vi "text_transceiver_sim.vi"() -> ()   [LabVIEW 2024]
uses:
  <vilib>/addons/Modulation/Digital/Channel Coding/MT Convolutional Encoder (Rate).vi
  <vilib>/Analysis/2dsp.llb/Inverse Complex FFT.vi
  <vilib>/Analysis/2dsp.llb/Complex FFT.vi
  <vilib>/addons/Modulation/Digital/Support/Common/Validators/mod_Generate Bits Validate.vi
  <vilib>/addons/Modulation/Digital/General/subVIs/mod_Generate Bits Pattern.vi
  <vilib>/addons/Modulation/Analog/support/mod_Set Error Source.vi
  <vilib>/addons/Modulation/Digital/Support/Common/Validators/mod_Validate Bit Stream.vi
  <vilib>/addons/Modulation/Digital/Channel Coding/Convolutional codes/mod_Convolutional encoder.vi
  <vilib>/addons/Modulation/Digital/Support/Common/Validators/mod_Validate Number of Rows Columns.vi
  <vilib>/addons/Modulation/Digital/Channel Coding/Block codes/subVIs/mod_Buffer block code info.vi
  <vilib>/addons/Modulation/Digital/Interleaving/Block Interleaver/mod_Block Interleaver (Matrix).vi
  <vilib>/addons/Modulation/Digital/DeInterleaving/Block DeInterleaver/mod_Block DeInterleaver (Matrix).vi
  <vilib>/addons/Modulation/Digital/Channel Coding/Convolutional codes/subVIs/mod_Generate encoder tap connections.vi
  <vilib>/addons/Modulation/Digital/Channel Coding/Convolutional codes/subVIs/mod_Perform convolutional encoding.vi
  <vilib>/addons/Modulation/Digital/Channel Coding/Block codes/subVIs/mod_Buffer block code info (I8).vi
  <vilib>/addons/Modulation/Digital/Channel Coding/Convolutional codes/subVIs/mod_Generate valid reset (convolutional, I8).vi
  <vilib>/addons/Modulation/Digital/Channel Coding/Convolutional codes/subVIs/mod_Select known generator matrix.vi
  <vilib>/addons/Modulation/Digital/Support/Common/Validators/mod_Validate Convolutional Encoder prms.vi
  <vilib>/addons/Modulation/Digital/General/MT Map Bits to PSK Symbols.vi
  <vilib>/addons/Modulation/Digital/General/subVIs/mod_Generate Bits PN Sequence.vi
  <vilib>/addons/Modulation/Digital/General/MT Map Bits to QAM Symbols.vi
  <vilib>/addons/Modulation/Digital/General/MT Map PSK Symbols to Bits.vi
  <vilib>/addons/Modulation/Digital/Channel Coding/MT Convolutional Decoder (Viterbi Hard Decision, Rate).vi
  <vilib>/addons/Modulation/Digital/General/MT Map QAM Symbols to Bits.vi
  <vilib>/Analysis/NI_AALPro.lvlib
  <vilib>/addons/Modulation/niDMT.lvlib
panel:
  in  "Ts":dbl
  out "x*y 3":cdb[](array[numeric])
  out "Coarse estimate":dbl
  out "Fine freq est":dbl
  in  "Delay":i32
  in  "freq_offset":dbl
  out "coarse freq est":dbl
  out "Fine estimate":i32
  out "Wifi signal":cdb[](array[numeric])
  out "Wifi signal after coarse freq sync":cdb[](array[numeric])
  out "Channel Estimate":cdb[](array[numeric])
  out "Received Message":string
  out "message bitstream":i8[](array[numeric])
  out "Header and payload symbols concetanated":cdb[][](array[numeric])
  out "Pilot polarities":dbl[][](array[numeric])
  out "Header symbols":cdb[](array[numeric]) format="%.3f"
  out "0, 1":i16
  in  "bit order":enum16{"MSB first", "LSB first"}(ring)=enum."LSB first"
  out "Message Length (bits)":i32
  in  "text message":string
  out "LLTF":cdb[](array[numeric])
  out "LSTF":cdb[](array[numeric])
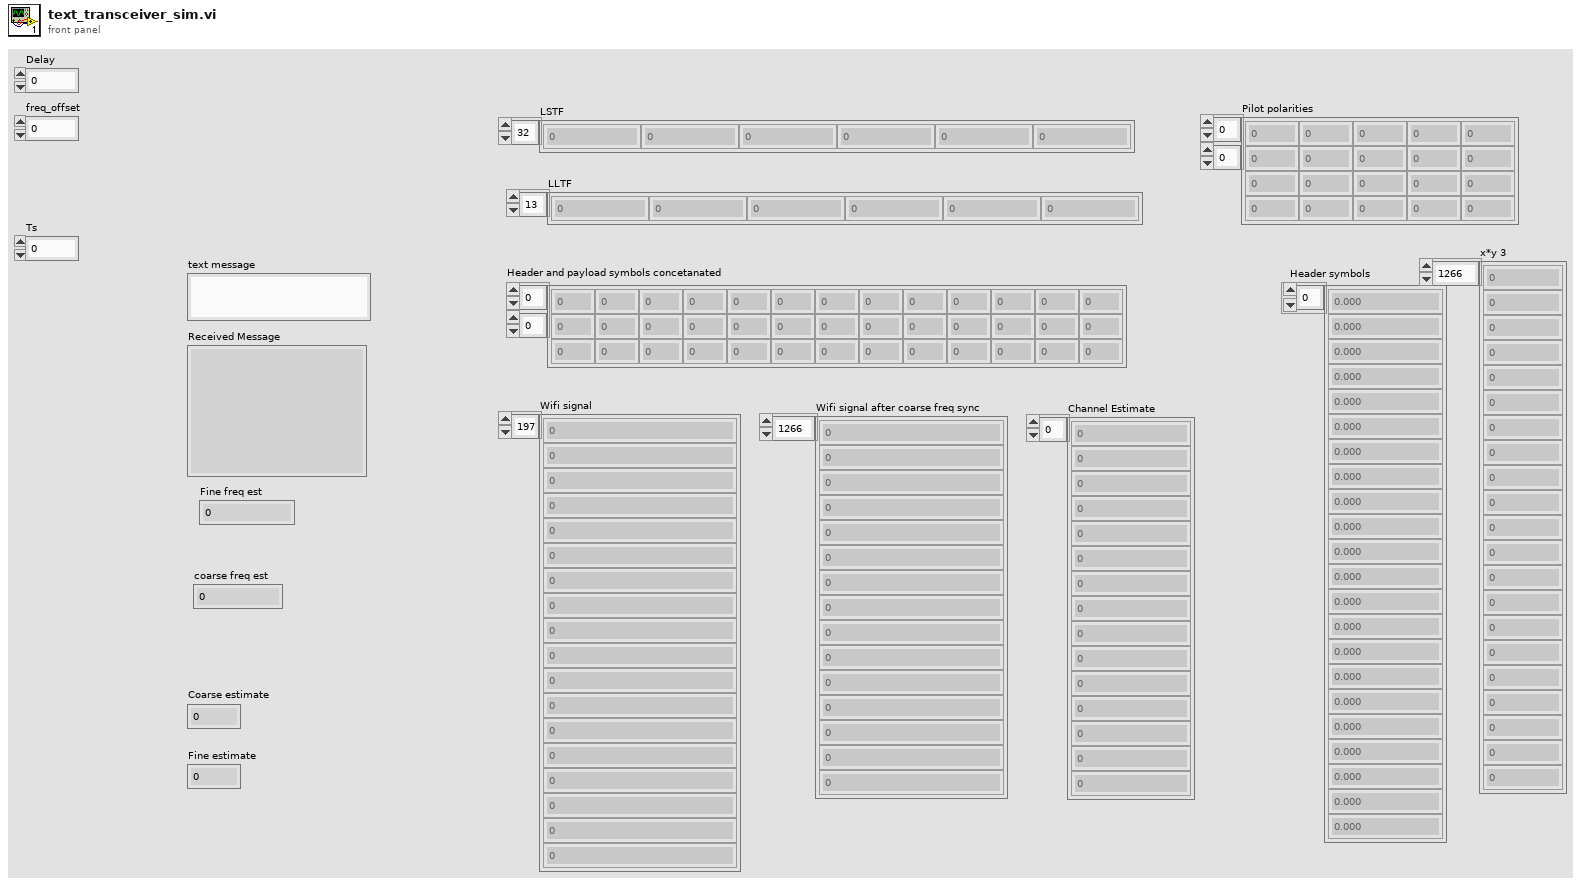
[diagram p1: front panel]
diagram:
  w9 = 80 ("dimension size")
  w35 = 8 ("y")
  w65 = 15 ("traceback depth (D)")
  w69 = cdb[] [0.7071067811865476+0.7071067811865476i, 0.7071067811865476-0.7071067811865476i, -0.7071067811865476+0.7071067811865476i, -0.7071067811865476-0.7071067811865476i]  # 4QAM MAP
  w77 = 15 ("traceback depth (D)")
  w101 = 48.0 ("y")
  w146 = cdb[] [0.7071067811865476+0.7071067811865476i, 0.7071067811865476-0.7071067811865476i, -0.7071067811865476+0.7071067811865476i, -0.7071067811865476-0.7071067811865476i]  # 4QAM MAP
  w175 = 0.0 ("element")
  w170 = 2.0 ("y")
  w169 = 1
  # "Delete preamble and S/P"
  # "Header symbols"
  # "BPSK demodulation"
  # "Payload symbols"
  # "# data carrying OFDM symbols"
  # "Service bits"
  # "# Pad bits"
  # "# service bits and tail bits"
  # "# data symbols"
  # "# data carrying OFDM symbols"
  # "# payload bits in an OFDM symbol"
  # "Interleaving"
  # "Pilot polarities"
  # "header OFDM sembolü"
  # "Wifi signal"
  # "Convolutional coding"
  # "Interleaving"
  # "scrambled pad bits"
  # "Tail"
  # "QPSK Modulation"
  # "BPSK modulation"
  # "Convolutional coding"
  # "Header and payload symbols concetanated"
  # "Header bits"
  # "Parity bit (even parity)"
  # "Tail bits"
  # "Length in bytes"
  # "Reserved bit"
  # "MCS"
  # "Num OFDM symbols\nHeader+data+padded data sym (pilot üretimi için bakıyoruz)"
  n1 = call "sub_Text_To_Bitstream.vi"("Packet\nMessage Length (bits)"=1 ("Packet\nMessage Length (bits)"), "text"="text message") -> ("File Length (bits)"=w115:i32, "message bitstream"=w122:i8[])  [unwired: 7 in, 1 out]
  "Message Length (bits)" <- w115
  "message bitstream" <- w122
  n2 = Add(x=w115, y=22) -> (x+y=w127:i32)
  n3 = Divide(x=w115, y=8.0) -> (x/y=w166:dbl)
  n4 = Add(x=w115, y=22) -> (x+y=w125:i32)
  n5 = Divide(x=w125, y=48) -> (x/y=w123:dbl)
  n6 = call <vilib>:"mod_Number to Bits.vi"("number of bits"=12, "bit order"="bit order", "Number"=w166) -> ("bits"=w161:i8[])  [unwired: 8 in]
  n7 = Build Array (concatenate)(i32[] [0, 0, 1, 0], i32[] [0], w161, i32[] [0, 0, 0, 0, 0, 0]) -> (w155:i32[])
  n8 = Add Array Elements(numeric array=w155) -> (sum=w153:i32)
  n9 = Round Toward +Infinity(x=w123) -> (ceil(x): smallest int >= x=w107:dbl)
  n10 = Add(x=w115, y=16.0) -> (x+y=w109:dbl)
  n11 = Multiply(x=w107, y=48) -> (x*y=w129:dbl)
  n12 = Add(x=w107, y=1 ("value")) -> (x+y=w105:dbl)
  n13 = Subtract(x=w129, y=w127) -> (x-y=w114:dbl)
  n14 = Quotient & Remainder(x=w153, y=2) -> (x-y*floor(x/y)=w158:i32)  [unwired: 1 out]
  n15 = Equal?(x=w158, y=1) -> (x = y?=w156:bool)
  n16 = Add(x=w114, y=6.0) -> (x+y=w112:dbl)
  n17 = Boolean To (0,1)(Boolean=w156) -> (0, 1=w152:i16)
  "0, 1" <- w152
  n18 = Initialize Array(0.0 ("element"), w112) -> (w119:dbl[])
  n19 = Build Array (concatenate)(i32[] [0, 0, 0, 0, 0, 0, 0, 0, 0, 0, 0, 0, 0, 0, 0, 0], w122, w119) -> (w108:dbl[])
  n20 = Array Size(array=w108) -> (size(s)=w118:i32)
  n21 = call <vilib>:"MT Generate Bits.vi"("total bits (128)"=w105, "PN sequence order (9)"=9) -> ("output bit stream"=w181:i8[])  [unwired: 11 in, 2 out]
  n22 = Multiply(x=w181, y=w170) -> (x*y=w182:dbl[])
  n23 = Multiply(x=w181, y=w170) -> (x*y=w180:dbl[])
  n24 = Insert Into Array(array=w155, index=17, new element=w152) -> (w150:i32[])
  n25 = call <vilib>:"MT Generate Bits.vi"("total bits (128)"=w118) -> ("output bit stream"=w117:i8[])  [unwired: 12 in, 2 out]
  n26 = Subtract(x=w180, y=w169) -> (x-y=w178:dbl[])
  n27 = Subtract(x=w169, y=w182) -> (x-y=w179:dbl[])
  n28 = Exclusive Or(1:w117, 2:w108) -> (0:w111:i32[])
  n29 = Build Array(w179, w179, w179, w178) -> (w177:dbl[][])
  n30 = call-poly <vilib>:"MT Convolutional Encode.vi"("input bit stream"=w150, "rate (k/n)"=enum16{"1/2", "1/3", "1/4", "2/3", "3/4"}."1/2") -> ("output bit stream"=w132:i8[])  [unwired: 11 in, 2 out]
  n31 = Transpose 2D Array(2D array=w177) -> (transposed array=w136:dbl[][])
  "Pilot polarities" <- w136
  n32 = call <vilib>:"MT Block Interleave (Matrix).vi"("data in"=w132, "number of rows"=16, "number of columns"=3) -> ("data out"=w131:i32[])  [unwired: 11 in, 1 out]
  n33 = Replace Array Subset(array=w111, new element=i32[] [0, 0, 0, 0, 0, 0], index=w109) -> (w104:i32[])
  n34 = call-poly <vilib>:"MT Map Bits to Symbols.vi"("input bit stream"=w131, "symbol map"=cdb[] [1.0+0.0i, -1.0+0.0i]) -> ("symbols"=w141:cdb[])  [unwired: 12 in, 1 out]
  "Header symbols" <- w141
  n35 = call-poly <vilib>:"MT Convolutional Encode.vi"("input bit stream"=w104, "rate (k/n)"=enum16{"1/2", "1/3", "1/4", "2/3", "3/4"}."1/2") -> ("output bit stream"=w103:i8[])  [unwired: 11 in, 2 out]
  n36 = Array Size(array=w103) -> (size(s)=w138:i32)
  n37 = call <vilib>:"MT Block Interleave (Matrix).vi"("data in"=w103, "number of rows"=16, "number of columns"=3) -> ("data out"=w137:i32[])  [unwired: 11 in, 1 out]
  n38 = for {
    N: w138 -> [_]
    tunnel: [w210] -> _ mode=indexing
    i -> [w214]
    n39 = Initialize Array(0.0 ("element"), 0 ("dimension size")) -> (w213:dbl[])
    n40 = Insert Into Array(array=w213, new element=w214) -> (w210:dbl[])  [unwired: 1 in]
  }
  n41 = call-poly <vilib>:"MT Map Bits to Symbols.vi"("input bit stream"=w137, "symbol map"=w146) -> ("symbols"=w145:cdb[])  [unwired: 12 in, 1 out]
  n42 = Array Size(array=w145) -> (size(s)=w144:i32)
  n43 = Divide(x=w144, y=w101) -> (x/y=w100:dbl)
  n44 = Reshape Array(w145, w100, w101) -> (w99:cdb[][])
  n45 = Build Array (concatenate)(w141, w99) -> (w102:cdb[][])
  "Header and payload symbols concetanated" <- w102
  n46 = Initialize Array(w175, w175, w175) -> (w174:dbl[][])
  n47 = Initialize Array(cdb 0.0+0.0i ("element"), 64 ("dimension size")) -> (w171:cdb[])
  n48 = for {
    tunnel: w102 -> [w231] mode=indexing
    tunnel: w136 -> [w230] mode=indexing
    shift-right: [w228] -> w140
    shift-left: w174 -> [w229]
    tunnel: w171 -> [w221]
    # "Concatenating OFDM symbols"
    # "CP insertion"
    # "IFFT"
    # "Zero padding"
    # "Pilot insertion"
    n49 = Add(x=i32[] [-21, -7, 7, 21], y=26.0) -> (x+y=w232:dbl[])
    n50 = for {
      tunnel: w232 -> [w238] mode=indexing
      shift-right: [w236] -> w226
      shift-left: w231 -> [w237]
      tunnel: w230 -> [w235] mode=indexing
      n51 = Insert Into Array(array=w237, index=w238, new element=w235) -> (w236:cdb[])
    }
    n52 = Split 1D Array(array=w226, index=26) -> (first subarray=w224:cdb[], second subarray=w223:cdb[])
    n53 = Replace Array Subset(array=w221, new element #1=w224, index #1=6 ("index"), new element #2=w223, index #2=33 ("index")) -> (w218:cdb[])
    n54 = call-poly <vilib>:"Inverse FFT.vi"("shift?"=TRUE, "FFT {X}"=w218) -> ("X"=w215:cdb[])  [unwired: 8 in, 1 out]
    n55 = Delete From Array(array=w215, length=16) -> (deleted portion=w216:cdb[])  [unwired: 1 in, 1 out]
    n56 = Build Array (concatenate)(w216, w215) -> (w217:cdb[])
    n57 = Build Array (concatenate)(w229, w217) -> (w228:cdb[][])
  }
  n58 = Initialize Array(cdb 0.0+0.0i ("element"), 64 ("dimension size")) -> (w207:cdb[])
  n59 = Divide(x=13.0, y=6.0) -> (x/y=w196:dbl)
  n60 = Square Root(x=w196) -> (sqrt(x)=w195:dbl)
  n61 = Replace Array Subset(array=w207, new element=cdb[] [0.0+0.0i, 0.0+0.0i, 1.0+1.0i, 0.0+0.0i, 0.0+0.0i, 0.0+0.0i, -1.0-1.0i, 0.0+0.0i, 0.0+0.0i, 0.0+0.0i, 1.0+1.0i, 0.0+0.0i, 0.0+0.0i, 0.0+0.0i, -1.0-1.0i, 0.0+0.0i, 0.0+0.0i, 0.0+0.0i, -1.0-1.0i, 0.0+0.0i, 0.0+0.0i, 0.0+0.0i, 1.0+1.0i, 0.0+0.0i, 0.0+0.0i, 0.0+0.0i, 0.0+0.0i, 0.0+0.0i, 0.0+0.0i, 0.0+0.0i, -1.0-1.0i, 0.0+0.0i, 0.0+0.0i, 0.0+0.0i, -1.0-1.0i, 0.0+0.0i, 0.0+0.0i, 0.0+0.0i, 1.0+1.0i, 0.0+0.0i, 0.0+0.0i, 0.0+0.0i, 1.0+1.0i, 0.0+0.0i, 0.0+0.0i, 0.0+0.0i, 1.0+1.0i, 0.0+0.0i, 0.0+0.0i, 0.0+0.0i, 1.0+1.0i, 0.0+0.0i, 0.0+0.0i], index=6) -> (w194:cdb[])
  n62 = Multiply(x=w194, y=w195) -> (x*y=w193:cdb[])
  n63 = Build Array (concatenate)(w193, w193) -> (w202:cdb[])
  n64 = Reshape Array(w202, 2 ("dimension size"), 64 ("dimension size")) -> (w201:cdb[][])
  n65 = for {
    tunnel: w201 -> [w244] mode=indexing
    tunnel: [w240] -> w200 mode=indexing
    n66 = call-poly <vilib>:"Inverse FFT.vi"("shift?"=TRUE, "FFT {X}"=w244) -> ("X"=w241:cdb[])  [unwired: 8 in, 1 out]
    n67 = Delete From Array(array=w241, length=16) -> (deleted portion=w242:cdb[])  [unwired: 1 in, 1 out]
    n68 = Build Array (concatenate)(w242, w241) -> (w240:cdb[])
  }
  n69 = Initialize Array(cdb 0.0+0.0i ("element"), 64 ("dimension size")) -> (w190:cdb[])
  n70 = Replace Array Subset(array=w190, new element=i32[] [1, 1, -1, -1, 1, 1, -1, 1, -1, 1, 1, 1, 1, 1, 1, -1, -1, 1, 1, -1, 1, -1, 1, 1, 1, 1, 0, 1, -1, -1, 1, 1, -1, 1, -1, 1, -1, -1, -1, -1, -1, 1, 1, -1, -1, 1, -1, 1, -1, 1, 1, 1, 1], index=6) -> (w95:cdb[])
  n71 = call-poly <vilib>:"Inverse FFT.vi"("shift?"=TRUE ("shift? 3"), "FFT {X}"=w95) -> ("X"=w187:cdb[])  [unwired: 8 in, 1 out]
  n72 = Build Array (concatenate)(w187, w187, w187) -> (w186:cdb[])
  n73 = Array Size(array=w140) -> (size(s)=w139:i32[])
  n74 = Split 1D Array(array=w186, index=32) -> (second subarray=w96:cdb[])  [unwired: 1 out]
  "LLTF" <- w96
  n75 = Multiply Array Elements(1:w139) -> (0:w148:i32)
  n76 = Reshape Array(w200, 160 ("dimension size")) -> (w14:cdb[])
  "LSTF" <- w14
  n77 = Initialize Array(0.0 ("element"), "Delay") -> (w15:dbl[])
  n78 = Reshape Array(w140, w148) -> (w135:cdb[])
  n79 = Build Array (concatenate)(w15, w14, w96, w135) -> (w1:cdb[])
  "Wifi signal" <- w1
  n80 = Array Size(array=w1) -> (size(s)=w29:i32)
  n81 = for {
    N: w29 -> [_]
    tunnel: [w245] -> w21 mode=indexing
    i -> [w245]
  }
  n82 = Multiply(x=2.0, y=3.141592653589793) -> (x*y=w25:dbl)
  n83 = Multiply(x=cdb 0.0+1.0i, y="Ts") -> (x*y=w24:cdb)
  n84 = Multiply(x=w24, y=w25) -> (x*y=w23:cdb)
  n85 = Multiply(x="freq_offset", y=w23) -> (x*y=w20:cdb)
  n86 = Multiply(x=w21, y=w20) -> (x*y=w19:cdb[])
  n87 = Exponential(1:w19) -> (0:w18:cdb[])
  n88 = Multiply(x=w18, y=w1) -> (x*y=w12:cdb[])
  "x*y 3" <- w12
  n89 = call "Coarse Timing Synchronization.vi"("Array"=w12) -> ("Coarse packet est"=w30:dbl)  [unwired: 9 in, 1 out]
  "Coarse estimate" <- w30
  n90 = call "Coarse Frequency Synchronization.vi"("Ts"="Ts", "Numeric in"=w30, "Array in"=w12) -> ("Array out"=w97:cdb[], "coarse freq est"=→"coarse freq est":dbl)  [unwired: 7 in]
  "Wifi signal after coarse freq sync" <- w97
  n91 = call "Fine Timing Synchronization.vi"("Long Preamble"=w96, "Coarse packet est"=w30, "Frame after coarse freq sync"=w97) -> ("Fine packet est"=→"Fine estimate":dbl, "Frame after fine time sync"=w31:cdb[])  [unwired: 7 in]
  n92 = call "Fine Frequency Synchronization.vi"("Frame after fine time sync"=w31, "Ts"="Ts") -> ("Fine freq est"=→"Fine freq est":dbl, "Frame after fine freq sync"=w5:cdb[])  [unwired: 8 in]
  n93 = call "Channel Estimation.vi"("Half of LLTF"=w95, "Frame after fine freq sync in"=w5) -> ("Channel Estimate"=w3:cdb[])  [unwired: 9 in]
  "Channel Estimate" <- w3
  n94 = Delete From Array(array=w5, length=320, index=0) -> (array with subset deleted=w11:cdb[])  [unwired: 1 out]
  n95 = Array Size(array=w11) -> (size(s)=w8:i32)
  n96 = Divide(x=w8, y=w9) -> (x/y=w10:dbl)
  n97 = Reshape Array(w11, w10, w9) -> (w4:cdb[][])
  n98 = for {
    tunnel: w4 -> [w249] mode=indexing
    tunnel: [w251] -> w93 mode=indexing
    tunnel: w3 -> [w248]
    # "Zero pad removal"
    # "Pilot removal"
    # "CP removal"
    n99 = Delete From Array(array=w249, length=16, index=0) -> (array with subset deleted=w265:cdb[])  [unwired: 1 out]
    n100 = call-poly <vilib>:"FFT.vi"("FFT size"=64, "shift?"=TRUE, "X"=w265) -> ("FFT {X}"=w247:cdb[])  [unwired: 7 in, 1 out]
    n101 = Divide(x=w247, y=w248) -> (x/y=w246:cdb[])
    n102 = Array Subset(array=w246, index=6, length=26) -> (w259:cdb[])
    n103 = Array Subset(array=w246, index=33, length=26) -> (w260:cdb[])
    n104 = Build Array(w259, w260) -> (w254:cdb[][])
    n105 = Array Size(array=w254) -> (size(s)=w256:i32[])
    n106 = Multiply Array Elements(1:w256) -> (0:w255:i32)
    n107 = Reshape Array(w254, w255) -> (w252:cdb[])
    n108 = Add(x=i32[] [-21, -7, 7, 21], y=26.0) -> (x+y=w253:dbl[])
    n109 = for {
      tunnel: w253 -> [w273] mode=indexing
      shift-right: [w270] -> w251
      shift-left: w252 -> [w269]
      i -> [w271]
      n110 = Subtract(x=w273, y=w271) -> (x-y=w272:dbl)
      n111 = Delete From Array(array=w269, length=1, index=w272) -> (array with subset deleted=w270:cdb[])  [unwired: 1 out]
    }
  }
  n112 = Array Size(array=w93) -> (size(s)=w94:i32[])
  n113 = Multiply Array Elements(1:w94) -> (0:w92:i32)
  n114 = Reshape Array(w93, w92) -> (w47:cdb[])
  n115 = Delete From Array(array=w47, length=48, index=0) -> (deleted portion=w80:cdb[], array with subset deleted=w46:cdb[])
  n116 = call-poly <vilib>:"MT Map Symbols to Bits.vi"("symbols"=w46, "symbol map"=w69) -> ("output bit stream"=w45:i8[])  [unwired: 12 in, 1 out]
  n117 = call-poly <vilib>:"MT Map Symbols to Bits.vi"("symbols"=w80, "symbol map"=cdb[] [1.0+0.0i, -1.0+0.0i]) -> ("output bit stream"=w86:i8[])  [unwired: 12 in, 1 out]
  n118 = call <vilib>:"MT Block DeInterleave (Matrix).vi"("data in"=w45, "number of rows"=16, "number of columns"=3) -> ("data out"=w61:i32[])  [unwired: 11 in, 1 out]
  n119 = Array Size(array=w61) -> (size(s)=w53:i32)
  n120 = call <vilib>:"MT Block DeInterleave (Matrix).vi"("data in"=w86, "number of rows"=16, "number of columns"=3) -> ("data out"=w70:i32[])  [unwired: 11 in, 1 out]
  n121 = Multiply(x=w65, y=w53) -> (x*y=w66:i32)
  n122 = Array Size(array=w70) -> (size(s)=w50:i32)
  n123 = Multiply(x=w77, y=w50) -> (x*y=w78:i32)
  n124 = Initialize Array(0.0 ("element"), w66) -> (w63:dbl[])
  n125 = Build Array (concatenate)(w61, w63) -> (w62:dbl[])
  n126 = Initialize Array(0.0 ("element"), w78) -> (w75:dbl[])
  n127 = Multiply(x=0.5, y=w50) -> (x*y=w57:dbl)
  n128 = Build Array (concatenate)(w70, w75) -> (w74:dbl[])
  n129 = Multiply(x=0.5, y=w53) -> (x*y=w52:dbl)
  n130 = call-poly <vilib>:"MT Convolutional Decode.vi"("input bit stream"=w62, "traceback depth (D)"=w65, "rate (k/n)"=enum16{"1/2", "1/3", "1/4", "2/3", "3/4"}."1/2", "constraint length (K)"=3) -> ("output bit stream"=w59:i8[])  [unwired: 9 in, 2 out]
  n131 = call-poly <vilib>:"MT Convolutional Decode.vi"("input bit stream"=w74, "traceback depth (D)"=w77, "rate (k/n)"=enum16{"1/2", "1/3", "1/4", "2/3", "3/4"}."1/2", "constraint length (K)"=3) -> ("output bit stream"=w73:i8[])  [unwired: 9 in, 2 out]
  n132 = Array Subset(array=w59, index=0, length=w52) -> (w42:i8[])
  n133 = Array Size(array=w42) -> (size(s)=w44:i32)
  n134 = Array Subset(array=w73, index=0, length=w57) -> (w71:i8[])
  n135 = call <vilib>:"MT Generate Bits.vi"("total bits (128)"=w44) -> ("output bit stream"=w43:i8[])  [unwired: 12 in, 2 out]
  n136 = Array Subset(array=w71, index=5, length=12) -> (w81:i8[])
  n137 = Exclusive Or(1:w43, 2:w42) -> (0:w41:i8[])
  n138 = Equal?(x=w81, y=1.0) -> (x = y?=w82:bool[])
  n139 = Boolean Array To Number(Boolean array=w82) -> (number=w49:u32)
  n140 = Multiply(x=u32 8, y=w49) -> (x*y=w39:u32)
  n141 = Array Subset(array=w41, index=16, length=w39) -> (w38:i8[])
  n142 = Array Size(array=w38) -> (size(s)=w37:i32)
  n143 = Divide(x=w37, y=w35) -> (x/y=w36:dbl)
  n144 = Reshape Array(w38, w36, w35) -> (w34:i8[][])
  n145 = call "sub_Format Rx Data.vi"("Output Packet Array"=w34) -> ("Received Message"=→"Received Message":string)
